vi "Read Scalar Data.vi"(8 "error in (no error)":errorcluster, 9 "Values":dbl[](array[numeric]), 11 "Cluster":T1={"Name"="", "Data Type"=enum."<Null>", "session"=0, "Scalar Type"=enum."Standard", "Index"=0, "Length"=0, "attributes"=variant(refnum<k20> refnum), "default value"=variant(refnum<k20> refnum), "RegisterOffset"=0} {"Data Type" format="%.0x"}) -> (0 "error out":errorcluster, 1 "Values":dbl[](array[numeric]))   [LabVIEW 2020, in "FPGA Addon Engine.lvlib"]
uses:
  FPGA Addon Engine.lvlib
  APIs/FPGA Register IO/FPGA Register IO.lvlib
  4847d5d1-9440-40b6-92fb-832ff25a6fdc.vi
  7af18865-f61b-4feb-9d18-9890e31bbcd0.vi
  Submodules/Source/Types/PWM.Measure.Analog.Measurement.ctl
  Submodules/Source/Types/PWM.Measure.Digital.Measurement.ctl
  0afef490-ebe9-4ede-9c00-a8227e1e55c9.vi
  faad099b-d847-4a24-8cce-cf54877fb1f0.vi
  Submodules/Source/Types/QuadratureEncoder.Measure.Digital.Measurement.ctl
  Submodules/Source/Types/Static.Measure.Digital.Measurement.ctl
  <vilib>/fxp/LVFixedPointRepBitsTypeDef.ctl
  <vilib>/fxp/LVFixedPointRepRangeTypeDef.ctl
  APIs/FPGA Register IO/TypeDefs/FXP Configuration.ctl
  APIs/FPGA Register IO/Read Methods/Read Data Register/Instances/Read I8.vi
  APIs/FPGA Register IO/Read Methods/Read Data Register/Instances/Read I16.vi
  APIs/FPGA Register IO/Read Methods/Read Data Register/Instances/Read I32.vi
  APIs/FPGA Register IO/Read Methods/Read Data Register/Instances/Read I64.vi
  APIs/FPGA Register IO/Read Methods/Read Data Register/Instances/Read U8.vi
  APIs/FPGA Register IO/Read Methods/Read Data Register/Instances/Read U16.vi
  APIs/FPGA Register IO/Read Methods/Read Data Register/Instances/Read U32.vi
  APIs/FPGA Register IO/Read Methods/Read Data Register/Instances/Read U64.vi
  APIs/FPGA Register IO/Read Methods/Read Data Register/Instances/Read SGL.vi
  APIs/FPGA Register IO/Read Methods/Read Data Register/Instances/Read Boolean.vi
  APIs/FPGA Register IO/Read Methods/Read Data Register/Instances/Read FXP.vi
  Types/Register Settings.ctl
  Addon Shared/Types/Scalar Type.ctl
  Addon Shared/FPGA Addon Shared.lvlib
  Addon Shared/Types/FPGA Addon Data Type.ctl
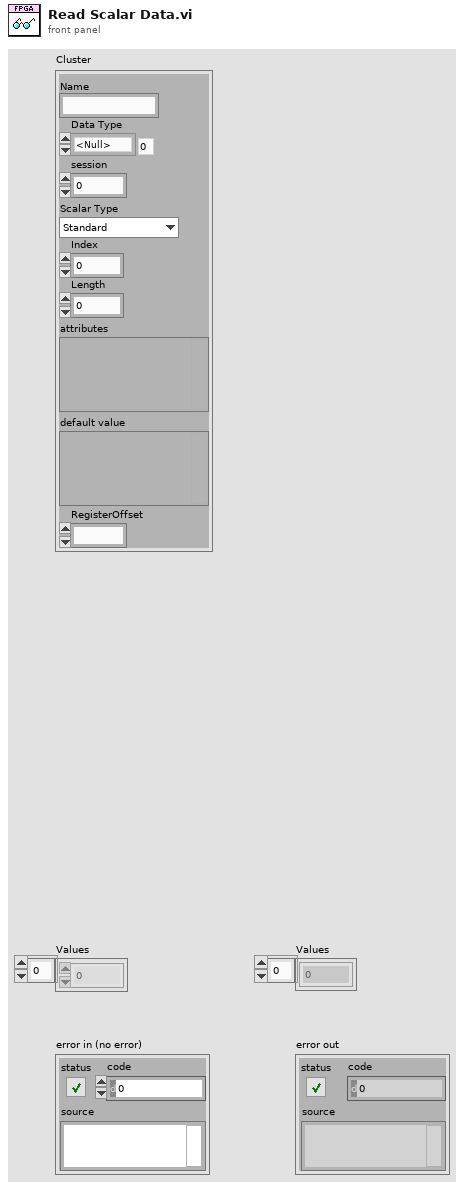
[diagram p1: front panel]
types:
  T1 = typedef "FPGA Addon Engine.lvlib/Register Settings.ctl" = cluster{"Name":string, "Data Type":T2, "session":u32, "Scalar Type":T3, "Index":i32, "Length":i32, "attributes":variant, "default value":variant, "RegisterOffset":u32}
  T2 = typedef "FPGA Addon Shared.lvlib/FPGA Addon Data Type.ctl" = enum8{"<Null>", "I8", "I16", "I32", "I64", "U8", "U16", "U32", "U64", "SGL", "Boolean", "Analog PWM In Settings", "Analog PWM In", "Digital PWM In Settings", "Digital PWM In", "Digital PWM Out", "Sine Out", "FXP", "FXP+/-24.5", "FXP+/-16.5", "FXP+/-32.8", "FXP+/-64.32", "FXP+/-16.7", "FXP+/-20.5", "FXP+/-27.5", "FXP+/-32.16", "FXP+16.3", "FXP+18.3", "Digital Static In", "Digital Static Out", "Digital Static In Settings", "Digital WSS Out", "Quad Encoder Settings", "Quad Encoder In", "Group"}
  T3 = typedef "FPGA Addon Shared.lvlib/Scalar Type.ctl" = enum16{"Standard", "Bitpacked"}
  T4 = typedef "FPGA Register IO.lvlib/FXP Configuration.ctl" = cluster{"FXP Representation":T5, "FXP Range":T6}
  T5 = typedef "LVFixedPointRepBitsTypeDef.ctl" = cluster{"Signed":bool, "Word Length":u32, "Integer Word Length":i32}
  T6 = typedef "LVFixedPointRepRangeTypeDef.ctl" = cluster{"Range Min":dbl, "Range Max":dbl, "Delta":dbl}
  T7 = typedef "Speciality FPGA IO.lvlib/Static.Measure.Digital.Measurement.ctl" = cluster{"STATE":bool}
  T8 = typedef "Speciality FPGA IO.lvlib/PWM.Measure.Analog.Measurement.ctl" = cluster{"ACTIVE TICKS":u32, "INACTIVE TICKS":u32, "ACQ TICKS":u32, "ACTIVE VOLTAGE":fxp<+/-,32,8>, "INACTIVE VOLTAGE":fxp<+/-,32,8>}
  T9 = typedef "Speciality FPGA IO.lvlib/PWM.Measure.Digital.Measurement.ctl" = cluster{"ACTIVE TICKS":u32, "INACTIVE TICKS":u32, "ACQ TICKS":u32}
  T10 = typedef "Speciality FPGA IO.lvlib/QuadratureEncoder.Measure.Digital.Measurement.ctl" = cluster{"POSITION":i32}
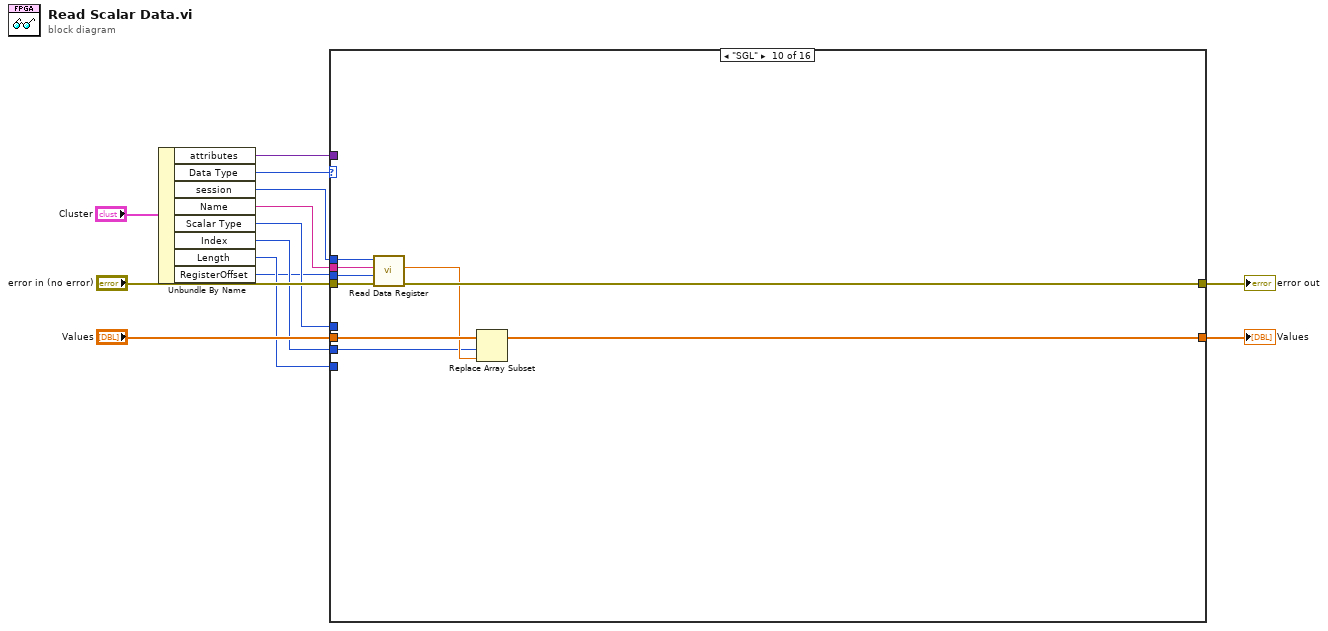
[diagram p0: block diagram]
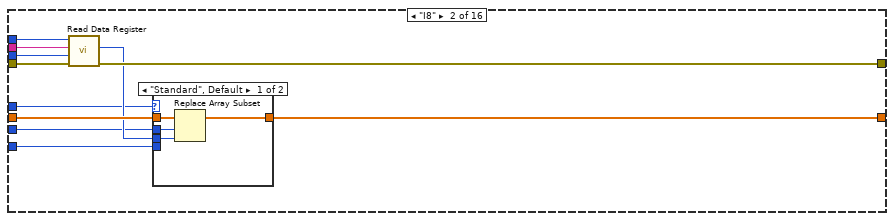
[diagram p3: hidden frame]
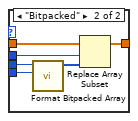
[diagram p4: hidden frame]
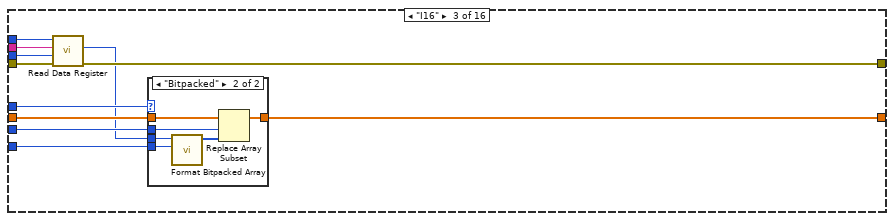
[diagram p5: hidden frame]
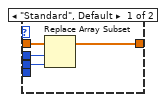
[diagram p6: hidden frame]
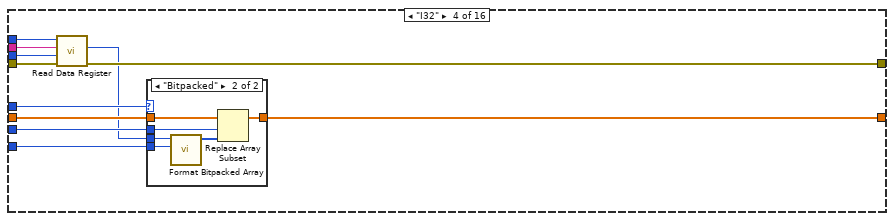
[diagram p7: hidden frame]
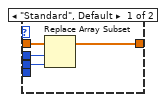
[diagram p8: hidden frame]
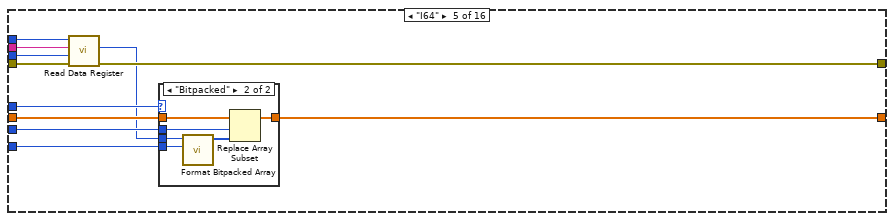
[diagram p9: hidden frame]
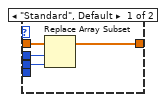
[diagram p10: hidden frame]
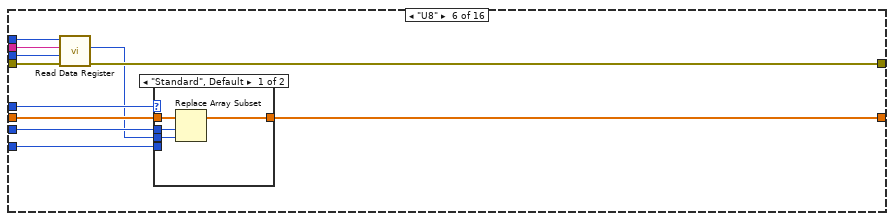
[diagram p11: hidden frame]
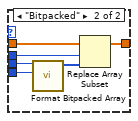
[diagram p12: hidden frame]
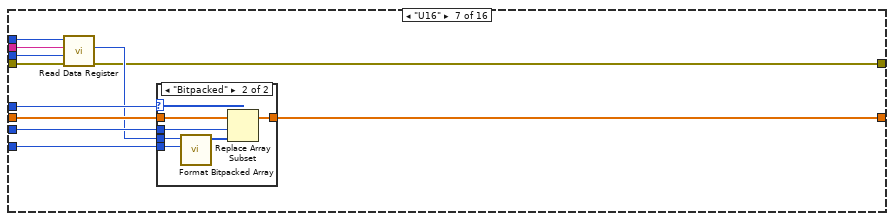
[diagram p13: hidden frame]
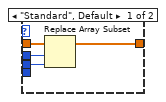
[diagram p14: hidden frame]
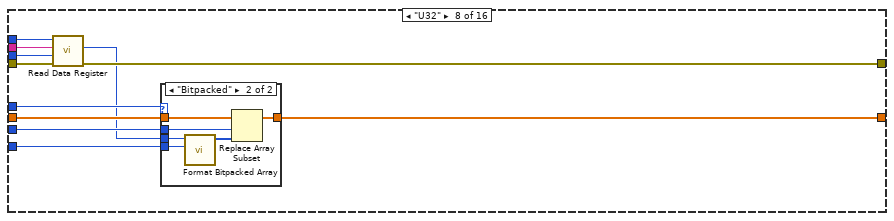
[diagram p15: hidden frame]
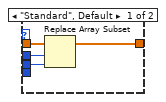
[diagram p16: hidden frame]
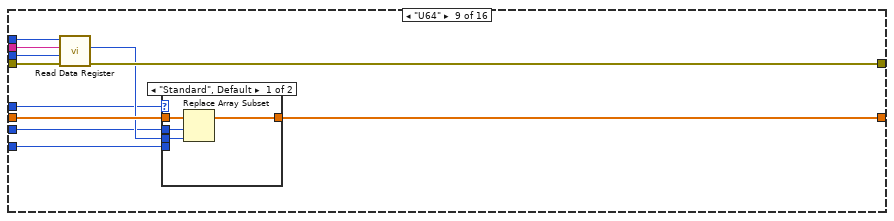
[diagram p17: hidden frame]
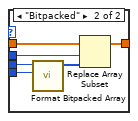
[diagram p18: hidden frame]
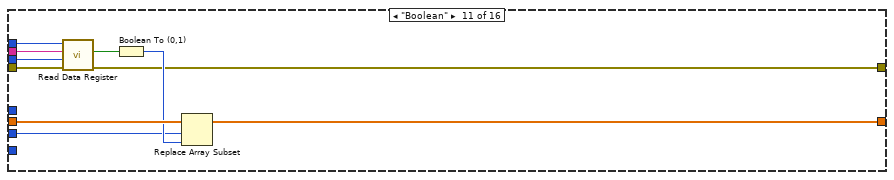
[diagram p19: hidden frame]
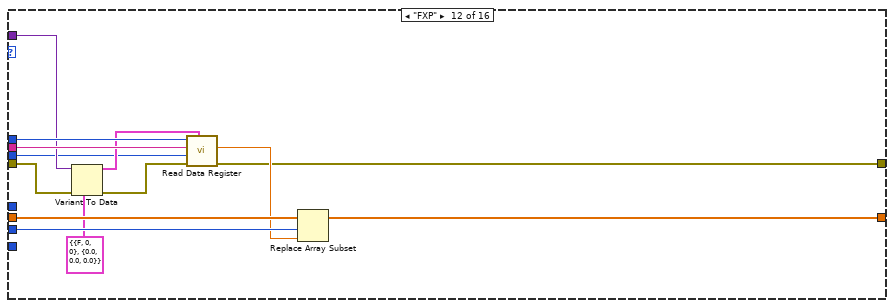
[diagram p20: hidden frame]
diagram:
  n1 = Unbundle By Name("Cluster") -> ("attributes"=w2:variant, "Data Type"=w8:T2, "session"=w7:u32, "Name"=w6:string, "Scalar Type"=w5:T3, "Index"=w4:i32, "Length"=w3:i32, "RegisterOffset"=w1:u32)
  n2 = case shown="\"SGL\"" w8 {
    tunnel: "error in (no error)" -> [w15 w23 w44 w63 w84 w105 w126 w149 w170 w190 w199 w207 w223 w232 w267 w300]
    tunnel: [w15 w21 w43 w62 w83 w104 w123 w148 w169 w189 w198 w209 w216 w231 w266 w299] -> w12
    tunnel: w3 -> [_ w25 w46 w66 w88 w109 w131 w150 w173 _ _ _ _ _ _ _]
    tunnel: w4 -> [_ w18 w40 w64 w85 w106 w127 w145 w165 w187 w195 w213 w224 w233 w269 w301]
    tunnel: w5 -> [_ w19 w41 w65 w86 w107 w128 w146 w166 _ _ _ _ _ _ _]
    tunnel: "Values" -> [w14 w26 w47 w68 w89 w110 w130 w152 w172 w192 w202 w215 w226 w244 w276 w304]
    tunnel: [w14 w24 w45 w67 w87 w108 w129 w151 w171 w191 w200 w214 w225 w243 w275 w303] -> w9
    tunnel: w6 -> [_ w22 w42 w60 w81 w102 w125 w147 w167 w186 w196 w212 w219 w230 w263 w295]
    tunnel: w7 -> [_ w17 w38 w59 w80 w101 w122 w143 w164 w185 w194 w211 w222 w229 w264 w296]
    tunnel: w2 -> [_ _ _ _ _ _ _ _ _ _ _ w208 _ _ _ _]
    tunnel: w1 -> [_ w16 w37 w58 w79 w100 w121 w142 w163 w184 w193 w203 _ _ _ _]
    frame "<Null>", Default {
    }
    frame "I8" {
      n3 = call-poly "Read Data Register.vi"("error in"=w23, "RegisterOffset"=w16, "register name"=w22, "session in"=w17) -> ("error out"=w21:errorcluster, "value out"=w20:i8)  [unwired: 5 in, 1 out]
      n4 = case shown="\"Standard\", Default" w19 {
        tunnel: w26 -> [w30 w35]
        tunnel: [w29 w34] -> w24
        tunnel: w25 -> [_ w36]
        tunnel: w20 -> [w27 w32]
        tunnel: w18 -> [w28 w31]
        frame "Standard", Default {
          n5 = Replace Array Subset(array=w30, new element=w27, index=w28) -> (w29:dbl[])
        }
        frame "Bitpacked" {
          n6 = call "Format Bitpacked Array.vi"("Length"=w36, "Value"=w32) -> ("Array"=w33:i16[])  [unwired: 9 in]
          n7 = Replace Array Subset(array=w35, new element=w33, index=w31) -> (w34:dbl[])
        }
      }
    }
    frame "I16" {
      n8 = call-poly "Read Data Register.vi"("error in"=w44, "RegisterOffset"=w37, "register name"=w42, "session in"=w38) -> ("error out"=w43:errorcluster, "value out"=w39:i16)  [unwired: 5 in, 1 out]
      n9 = case shown="\"Bitpacked\"" w41 {
        tunnel: w47 -> [w51 w56]
        tunnel: [w50 w55] -> w45
        tunnel: w39 -> [w49 w52]
        tunnel: w40 -> [w48 w53]
        tunnel: w46 -> [_ w57]
        frame "Standard", Default {
          n10 = Replace Array Subset(array=w51, new element=w49, index=w48) -> (w50:dbl[])
        }
        frame "Bitpacked" {
          n11 = call "Format Bitpacked Array.vi"("Length"=w57, "Value"=w52) -> ("Array"=w54:i16[])  [unwired: 9 in]
          n12 = Replace Array Subset(array=w56, new element=w54, index=w53) -> (w55:dbl[])
        }
      }
    }
    frame "I32" {
      n13 = call-poly "Read Data Register.vi"("error in"=w63, "RegisterOffset"=w58, "register name"=w60, "session in"=w59) -> ("error out"=w62:errorcluster, "value out"=w61:i32)  [unwired: 5 in, 1 out]
      n14 = case shown="\"Bitpacked\"" w65 {
        tunnel: w68 -> [w72 w76]
        tunnel: [w71 w75] -> w67
        tunnel: w61 -> [w70 w78]
        tunnel: w64 -> [w69 w73]
        tunnel: w66 -> [_ w77]
        frame "Standard", Default {
          n15 = Replace Array Subset(array=w72, new element=w70, index=w69) -> (w71:dbl[])
        }
        frame "Bitpacked" {
          n16 = call "Format Bitpacked Array.vi"("Length"=w77, "Value"=w78) -> ("Array"=w74:i16[])  [unwired: 9 in]
          n17 = Replace Array Subset(array=w76, new element=w74, index=w73) -> (w75:dbl[])
        }
      }
    }
    frame "I64" {
      n18 = call-poly "Read Data Register.vi"("error in"=w84, "RegisterOffset"=w79, "register name"=w81, "session in"=w80) -> ("error out"=w83:errorcluster, "value out"=w82:i64)  [unwired: 5 in, 1 out]
      n19 = case shown="\"Bitpacked\"" w86 {
        tunnel: w89 -> [w93 w97]
        tunnel: [w92 w96] -> w87
        tunnel: w82 -> [w91 w99]
        tunnel: w85 -> [w90 w94]
        tunnel: w88 -> [_ w98]
        frame "Standard", Default {
          n20 = Replace Array Subset(array=w93, new element=w91, index=w90) -> (w92:dbl[])
        }
        frame "Bitpacked" {
          n21 = call "Format Bitpacked Array.vi"("Length"=w98, "Value"=w99) -> ("Array"=w95:i16[])  [unwired: 9 in]
          n22 = Replace Array Subset(array=w97, new element=w95, index=w94) -> (w96:dbl[])
        }
      }
    }
    frame "U8" {
      n23 = call-poly "Read Data Register.vi"("error in"=w105, "RegisterOffset"=w100, "register name"=w102, "session in"=w101) -> ("error out"=w104:errorcluster, "value out"=w103:u8)  [unwired: 5 in, 1 out]
      n24 = case shown="\"Standard\", Default" w107 {
        tunnel: w110 -> [w114 w119]
        tunnel: [w113 w118] -> w108
        tunnel: w109 -> [_ w120]
        tunnel: w106 -> [w112 w116]
        tunnel: w103 -> [w111 w115]
        frame "Standard", Default {
          n25 = Replace Array Subset(array=w114, new element=w111, index=w112) -> (w113:dbl[])
        }
        frame "Bitpacked" {
          n26 = call "Format Bitpacked Array.vi"("Length"=w120, "Value"=w115) -> ("Array"=w117:i16[])  [unwired: 9 in]
          n27 = Replace Array Subset(array=w119, new element=w117, index=w116) -> (w118:dbl[])
        }
      }
    }
    frame "U16" {
      n28 = call-poly "Read Data Register.vi"("error in"=w126, "RegisterOffset"=w121, "register name"=w125, "session in"=w122) -> ("error out"=w123:errorcluster, "value out"=w124:u16)  [unwired: 5 in, 1 out]
      n29 = case shown="\"Bitpacked\"" w128 {
        tunnel: w130 -> [w135 w139]
        tunnel: [w134 w138] -> w129
        tunnel: w124 -> [w133 w141]
        tunnel: w127 -> [w132 w136]
        tunnel: w131 -> [_ w140]
        frame "Standard", Default {
          n30 = Replace Array Subset(array=w135, new element=w133, index=w132) -> (w134:dbl[])
        }
        frame "Bitpacked" {
          n31 = call "Format Bitpacked Array.vi"("Length"=w140, "Value"=w141) -> ("Array"=w137:i16[])  [unwired: 9 in]
          n32 = Replace Array Subset(array=w139, new element=w137, index=w136) -> (w138:dbl[])
        }
      }
    }
    frame "U32" {
      n33 = call-poly "Read Data Register.vi"("error in"=w149, "RegisterOffset"=w142, "register name"=w147, "session in"=w143) -> ("error out"=w148:errorcluster, "value out"=w144:u32)  [unwired: 5 in, 1 out]
      n34 = case shown="\"Bitpacked\"" w146 {
        tunnel: w152 -> [w156 w160]
        tunnel: [w155 w159] -> w151
        tunnel: w144 -> [w154 w162]
        tunnel: w145 -> [w153 w157]
        tunnel: w150 -> [_ w161]
        frame "Standard", Default {
          n35 = Replace Array Subset(array=w156, new element=w154, index=w153) -> (w155:dbl[])
        }
        frame "Bitpacked" {
          n36 = call "Format Bitpacked Array.vi"("Length"=w161, "Value"=w162) -> ("Array"=w158:i16[])  [unwired: 9 in]
          n37 = Replace Array Subset(array=w160, new element=w158, index=w157) -> (w159:dbl[])
        }
      }
    }
    frame "U64" {
      n38 = call-poly "Read Data Register.vi"("error in"=w170, "RegisterOffset"=w163, "register name"=w167, "session in"=w164) -> ("error out"=w169:errorcluster, "value out"=w168:u64)  [unwired: 5 in, 1 out]
      n39 = case shown="\"Standard\", Default" w166 {
        tunnel: w172 -> [w177 w181]
        tunnel: [w176 w180] -> w171
        tunnel: w168 -> [w175 w183]
        tunnel: w165 -> [w174 w178]
        tunnel: w173 -> [_ w182]
        frame "Standard", Default {
          n40 = Replace Array Subset(array=w177, new element=w175, index=w174) -> (w176:dbl[])
        }
        frame "Bitpacked" {
          n41 = call "Format Bitpacked Array.vi"("Length"=w182, "Value"=w183) -> ("Array"=w179:i16[])  [unwired: 9 in]
          n42 = Replace Array Subset(array=w181, new element=w179, index=w178) -> (w180:dbl[])
        }
      }
    }
    frame "SGL" {
      n43 = call-poly "Read Data Register.vi"("error in"=w190, "RegisterOffset"=w184, "register name"=w186, "session in"=w185) -> ("error out"=w189:errorcluster, "value out"=w188:sgl)  [unwired: 5 in, 1 out]
      n44 = Replace Array Subset(array=w192, new element=w188, index=w187) -> (w191:dbl[])
    }
    frame "Boolean" {
      n45 = call-poly "Read Data Register.vi"("error in"=w199, "RegisterOffset"=w193, "register name"=w196, "session in"=w194) -> ("error out"=w198:errorcluster, "value out"=w197:bool)  [unwired: 5 in, 1 out]
      n46 = Boolean To (0,1)(Boolean=w197) -> (0, 1=w201:i16)
      n47 = Replace Array Subset(array=w202, new element=w201, index=w195) -> (w200:dbl[])
    }
    frame "FXP" {
      n48 = Variant To Data(error in=w207, type=T4 {"FXP Representation"={"Signed"=FALSE, "Word Length"=0, "Integer Word Length"=0}, "FXP Range"={"Range Min"=0.0, "Range Max"=0.0, "Delta"=0.0}} ("FXP Configuration"), Variant=w208) -> (data=w204:T4, error out=w206:errorcluster)
      n49 = call-poly "Read Data Register.vi"("FXP Configuration"=w204, "error in"=w206, "RegisterOffset"=w203, "register name"=w212, "session in"=w211) -> ("error out"=w209:errorcluster, "DBL Value"=w210:dbl)  [unwired: 4 in, 1 out]
      n50 = Replace Array Subset(array=w215, new element=w210, index=w213) -> (w214:dbl[])
    }
    frame "Digital Static In" {
      n51 = call "Read Cluster Register.vim"("error in (no error)"=w223, "Cluster in (default value)"=T7 {"STATE"=FALSE}, "Cluster Name"=w219, "session in"=w222) -> ("error out"=w216:errorcluster, "Cluster out"=w221:T7)  [unwired: 4 in, 2 out]
      n52 = Unbundle By Name(w221) -> ("STATE"=w217:bool)
      n53 = Boolean To (0,1)(Boolean=w217) -> (0, 1=w218:i16)
      n54 = Replace Array Subset(array=w226, new element=w218, index=w224) -> (w225:dbl[])
    }
    frame "Analog PWM In" {
      w251 = 2.5000000292152436e-08 ("y")
      n55 = call "Read Cluster Register.vim"("error in (no error)"=w232, "Cluster in (default value)"=T8 {"ACTIVE TICKS"=0, "INACTIVE TICKS"=0, "ACQ TICKS"=0, "ACTIVE VOLTAGE"=0.0, "INACTIVE VOLTAGE"=0.0}, "Cluster Name"=w230, "session in"=w229) -> ("error out"=w231:errorcluster, "Cluster out"=w227:T8)  [unwired: 4 in, 2 out]
      n56 = Unbundle By Name(w227) -> ("ACTIVE TICKS"=w240:u32, "INACTIVE TICKS"=w239:u32, "ACQ TICKS"=w238:u32, "ACTIVE VOLTAGE"=w237:fxp<+/-,32,8>, "INACTIVE VOLTAGE"=w236:fxp<+/-,32,8>)
      n57 = Add(x=w240, y=w239) -> (x+y=w253:u32)
      n58 = Compound Arithmetic op=MULTIPLY(w253, w238, w251) -> (w254:dbl)
      n59 = Divide(x=w240, y=w253) -> (x/y=w247:dbl)
      n60 = Compound Arithmetic op=MULTIPLY(w240, w238, w251) -> (w252:dbl)
      n61 = Multiply(x=100.0, y=w247) -> (x*y=w246:dbl)
      n62 = Equal?(x=0.0, y=w254) -> (x = y?=w250:bool)
      n63 = Reciprocal(x=w254) -> (1/x=w255:dbl)
      n64 = case shown="False" w250 {
        tunnel: [w257 w261] -> w235
        tunnel: [w258 w261] -> w241
        tunnel: [w260 w261] -> w234
        tunnel: w254 -> [w260 _]
        tunnel: [w259 w261] -> w245
        tunnel: w252 -> [w259 _]
        tunnel: w246 -> [w258 _]
        tunnel: w255 -> [w257 _]
        tunnel: 0.0 ("x") -> [_ w261]
        frame False {
        }
        frame True {
        }
      }
      n65 = Build Array(w235, w234, w241, w245, w237, w236) -> (w242:dbl[])
      n66 = Replace Array Subset(array=w244, new element=w242, index=w233) -> (w243:dbl[])
    }
    frame "Digital PWM In" {
      w284 = 2.5000000292152436e-08 ("y")
      n67 = call "Read Cluster Register.vim"("error in (no error)"=w267, "Cluster in (default value)"=T9 {"ACTIVE TICKS"=0, "INACTIVE TICKS"=0, "ACQ TICKS"=0}, "Cluster Name"=w263, "session in"=w264) -> ("error out"=w266:errorcluster, "Cluster out"=w262:T9)  [unwired: 4 in, 2 out]
      n68 = Unbundle By Name(w262) -> ("ACTIVE TICKS"=w268:u32, "INACTIVE TICKS"=w272:u32, "ACQ TICKS"=w280:u32)
      n69 = Add(x=w268, y=w272) -> (x+y=w286:u32)
      n70 = Compound Arithmetic op=MULTIPLY(w286, w280, w284) -> (w287:dbl)
      n71 = Divide(x=w268, y=w286) -> (x/y=w279:dbl)
      n72 = Compound Arithmetic op=MULTIPLY(w268, w280, w284) -> (w285:dbl)
      n73 = Multiply(x=100.0, y=w279) -> (x*y=w278:dbl)
      n74 = Equal?(x=0.0, y=w287) -> (x = y?=w283:bool)
      n75 = Reciprocal(x=w287) -> (1/x=w288:dbl)
      n76 = case shown="True" w283 {
        tunnel: [w290 w294] -> w271
        tunnel: [w291 w294] -> w273
        tunnel: [w293 w294] -> w270
        tunnel: w287 -> [w293 _]
        tunnel: [w292 w294] -> w277
        tunnel: w285 -> [w292 _]
        tunnel: w278 -> [w291 _]
        tunnel: w288 -> [w290 _]
        tunnel: 0.0 ("x") -> [_ w294]
        frame False {
        }
        frame True {
        }
      }
      n77 = Build Array(w271, w270, w273, w277) -> (w274:dbl[])
      n78 = Replace Array Subset(array=w276, new element=w274, index=w269) -> (w275:dbl[])
    }
    frame "Quad Encoder In" {
      n79 = call "Read Cluster Register.vim"("error in (no error)"=w300, "Cluster in (default value)"=T10 {"POSITION"=0}, "Cluster Name"=w295, "session in"=w296) -> ("error out"=w299:errorcluster, "Cluster out"=w297:T10)  [unwired: 4 in, 2 out]
      n80 = Unbundle By Name(w297) -> ("POSITION"=w302:i32)
      n81 = Replace Array Subset(array=w304, new element=w302, index=w301) -> (w303:dbl[])
    }
  }
  "error out" <- w12
  "Values" <- w9
